vi "to string.vi"(8 "error in":errorcluster, 11 "SQLite configuration in":refnum<class "SQLite configuration.lvclass">) -> (0 "error out":errorcluster, 1 "data":string, 2 "version":string, 3 "SQLite configuration out":refnum<class "SQLite configuration.lvclass">)   [LabVIEW 2014, in "SQLite configuration.lvclass"]
doc: "Provides an interface for saving a module configuration to a file or other serialized data source. It is recommended that all children of this class store data in two sets--data required for its own initialization, and any data required for parent initialization--and that each implementation uses the <b>Call Parent Method</b> primitive to serialize parent information."
uses:
  SQLite configuration.lvclass
  SQLite configuration.lvclass/SQLite configuration.ctl
  current version.vi
  <vilib>/NI/Tag Bus Module Framework/module configuration/TBM module configuration.lvclass
  <vilib>/NI/Tag Bus Module Framework/channel/TBM channel.lvclass
  <vilib>/NI/Configuration Framework/serializable configuration/NISE_CEF_serializable configuration.lvclass
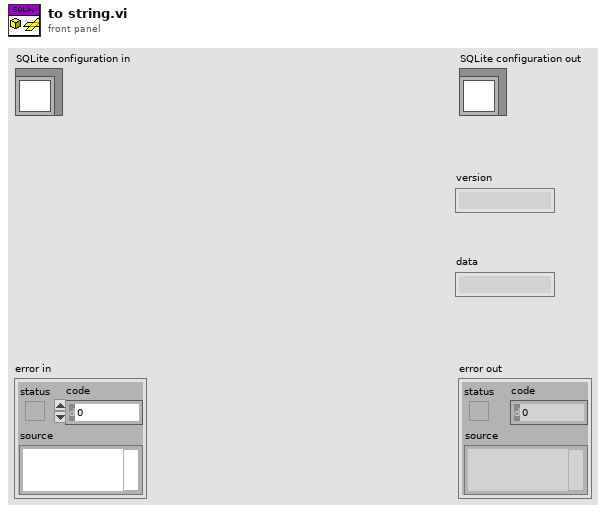
[diagram p1: front panel]
types:
  T1 = typedef "SQLite configuration.lvclass/Line.ctl" = cluster{"channel":refnum<class "TBM channel.lvclass">}
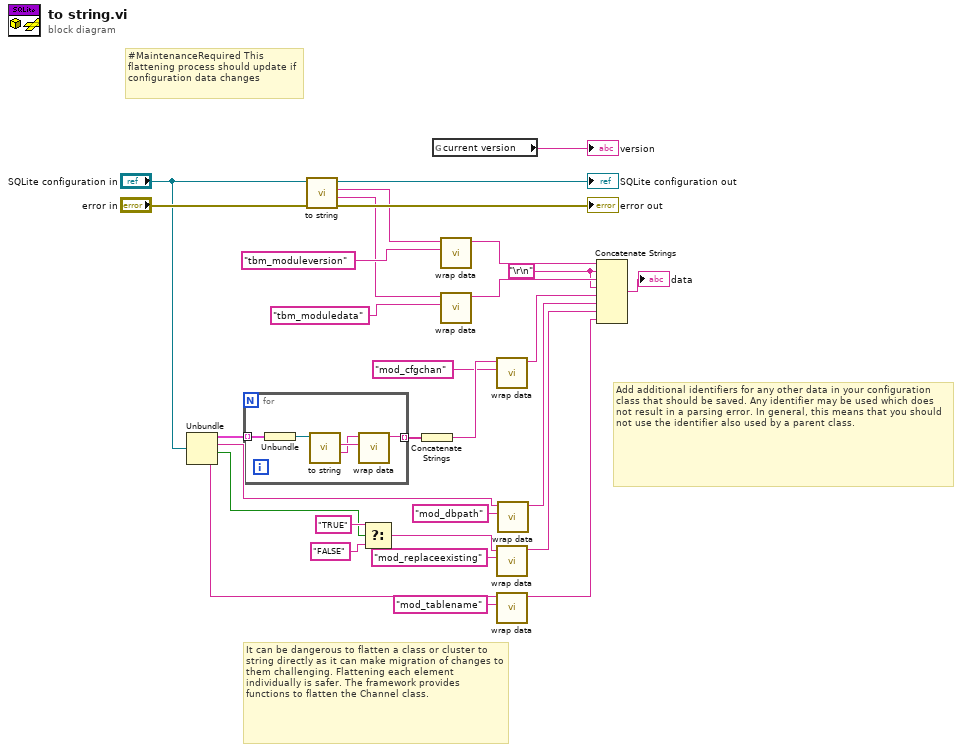
[diagram p0: block diagram]
diagram:
  w17 = "\r\n"
  # "It can be dangerous to flatten a class or cluster to string directly as it can make migration of changes to them challenging. Flattening each element individually is safer. The framework provides functions to flatten the Channel class."
  # "Add additional identifiers for any other data in your configuration class that should be saved. Any identifier may be used which does not result in a parsing error. In general, this means that you should not use the identifier also used by a parent class."
  # "#MaintenanceRequired This flattening process should update if configuration data changes"
  n1 = Unbundle("SQLite configuration in") -> (w16:T1[], w11:string, w2:bool, w9:string)
  n2 = for {
    tunnel: w16 -> [w35] mode=indexing
    tunnel: [w31] -> w15 mode=indexing
    n3 = Unbundle(w35) -> ("channel"=w34:refnum<class "TBM channel.lvclass">)
    n4 = call-dynamic "to string.vi"("channel in"=w34) -> ("channel data"=w32:string, "identifier"=w33:string)  [unwired: 7 in, 2 out]
    n5 = call <vilib>:"wrap data.vi"("identifier"=w33, "data to wrap"=w32) -> ("wrapped data"=w31:string)  [unwired: 9 in]
  }
  n6 = call-parent "to string.vi"("error in"="error in", "module configuration in"="SQLite configuration in") -> ("error out"=→"error out":errorcluster, "data"=w21:string, "version"=w22:string, "module configuration out"=→"SQLite configuration out":refnum<class "SQLite configuration.lvclass">)  [unwired: 6 in]
  n7 = Select(t="TRUE" ("identifier"), s=w2, f="FALSE" ("identifier")) -> (s? t:f=w1:string)
  n8 = Concatenate Strings(w15) -> (w14:string)
  n9 = global read "current version.vi" "current version"() -> (→"version":string)
  n10 = call <vilib>:"wrap data.vi"("identifier"="tbm_moduleversion" ("additional identifier"), "data to wrap"=w22) -> ("wrapped data"=w24:string)  [unwired: 9 in]
  n11 = call <vilib>:"wrap data.vi"("identifier"="tbm_moduledata" ("additional identifier"), "data to wrap"=w21) -> ("wrapped data"=w23:string)  [unwired: 9 in]
  n12 = call <vilib>:"wrap data.vi"("identifier"="mod_cfgchan", "data to wrap"=w14) -> ("wrapped data"=w18:string)  [unwired: 9 in]
  n13 = call <vilib>:"wrap data.vi"("identifier"="mod_replaceexisting", "data to wrap"=w1) -> ("wrapped data"=w6:string)  [unwired: 9 in]
  n14 = call <vilib>:"wrap data.vi"("identifier"="mod_tablename", "data to wrap"=w9) -> ("wrapped data"=w7:string)  [unwired: 9 in]
  n15 = call <vilib>:"wrap data.vi"("identifier"="mod_dbpath", "data to wrap"=w11) -> ("wrapped data"=w10:string)  [unwired: 9 in]
  n16 = Concatenate Strings(w24, w17, w23, w17, w18, w10, w6, w7) -> (→"data":string)
